vi "SlewRateLimiter_New.vi"(8 "Time":dbl=-1.0 format="%33.4f", 9 "InitialValue":dbl, 10 "NegativeRateLimit":dbl=1.0, 11 "PositiveRateLimit":dbl) -> (3 "out SLEW_RATE_LIMITER":T1 {"NegativeRateLimit" format="%13.5p"; "PrevTime" format="%30.5p"; "PrevValue" format="%13.5p"; "PositiveRateLimit" format="%13.5p"})   [LabVIEW 2019, in "Trajectory_Library.lvlib"]
doc: "Creates a new SlewRateLimiter data cluster with the given rate limit and initial value.\n\nThis set of functions limits the rate of change of an input value. Useful for implementing voltage, setpoint, and/or output ramps. A slew-rate limit is most appropriate when the quantity being controlled is a velocity or a voltage; when controlling a position, consider using a postion control algoritmn or trapezoid profile instead.\n\nInputs:\n - PositiveRateLimit -- The positive rate-of-change limit, in units per second. \n The value is expected to be >= 0.\n - NegativeRateLimit -- The negative rate-of-change limit, in units per second.\n The value is expected to be <= 0. If the value is not wired or is > 0 then\n the PositiveRateLimit * -1 is used. \n - initialValue -- The initial value of the input.\n \nOutputs:\n - out Slew Rate Limiter -- The initialized Slew Rate Limiter data cluster"
uses:
  Trajectory_Library.lvlib
  TypeDef/SLEW_RATE_LIMITER.ctl
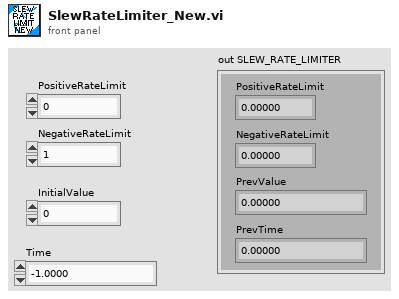
[diagram p1: front panel]
types:
  T1 = typedef "Trajectory_Library.lvlib/SLEW_RATE_LIMITER.ctl" = cluster{"PositiveRateLimit":dbl, "PrevValue":dbl, "PrevTime":dbl, "NegativeRateLimit":dbl}
  T2 = typedef "WPILib_Math.lvlib/SLEW_RATE_LIMITER.ctl" = cluster{"PositiveRateLimit":dbl, "PrevValue":dbl, "PrevTime":dbl, "NegativeRateLimit":dbl}
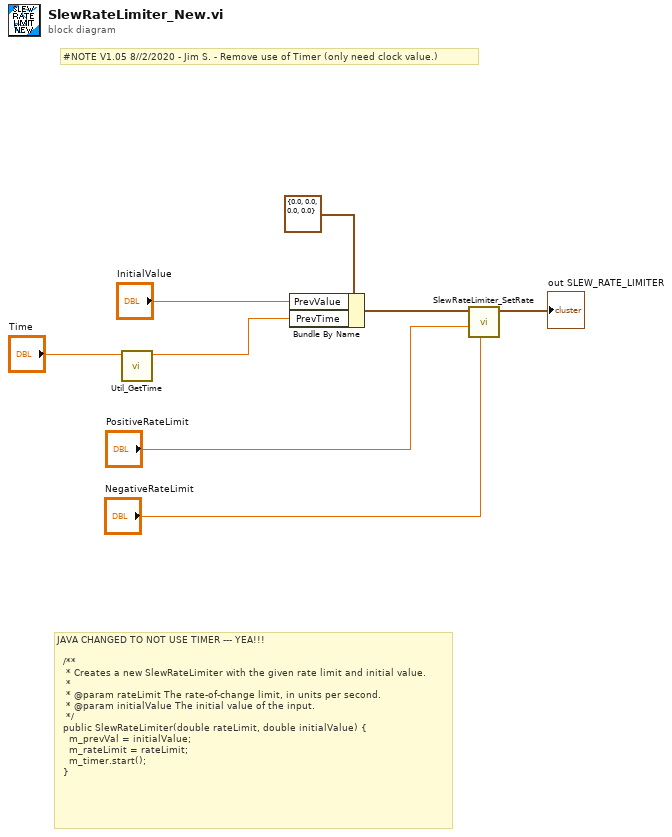
[diagram p0: block diagram]
diagram:
  # "#NOTE V1.05 8//2/2020 - Jim S. - Remove use of Timer (only need clock value.)"
  # "JAVA CHANGED TO NOT USE TIMER --- YEA!!!\n\n  /**\n   * Creates a new SlewRateLimiter with the given rate limit and initial value.\n   *\n   * @param rateLimit The rate-of-change limit, in units per second.\n   * @param initialValue The initial value of the input.\n   */\n  public SlewRateLimiter(double rateLimit, double initialValue) {\n    m_prevVal = initialValue;\n    m_rateLimit = rateLimit;\n    m_timer.start();\n  }"
  n1 = call "Util_GetTime.vi"("Pass_Through_Time"="Time") -> ("FPGA_Time_Seconds"=w6:dbl)  [unwired: 9 in, 1 out]
  n2 = Bundle By Name(cluster=T1 {"PositiveRateLimit"=0.0, "PrevValue"=0.0, "PrevTime"=0.0, "NegativeRateLimit"=0.0} ("out SLEW_RATE_LIMITER"), "PrevValue"="InitialValue", "PrevTime"=w6) -> (w4:T1)
  n3 = call "SlewRateLimiter_SetRate.vi"("NegativeRate"="NegativeRateLimit", "PositiveRate"="PositiveRateLimit", "in SLEW_RATE_LIMITER"=w4) -> ("out SLEW_RATE_LIMITER"=→"out SLEW_RATE_LIMITER":T2)  [unwired: 8 in]
